vi "Process.vi"(8 "error in":errorcluster, 11 "Plugin in":refnum<class "Nominal-Streamer.lvclass">) -> (0 "error out":errorcluster, 3 "Plugin out":refnum<class "Nominal-Streamer.lvclass">)   [LabVIEW 2020, in "Nominal-Streamer.lvlib" / "Nominal-Streamer.lvclass"]
doc: "Handles incoming data from NI FlexLogger (R) and forwards it to the async processing function."
uses:
  Nominal-Streamer.lvclass
  Nominal-Streamer.lvclass/Nominal-Streamer.ctl
  <vilib>/FlexLogger/SDK/PluginSDK.lvlibp/PEFClasses/SDK/Plugin/Plugin.lvclass
  async queue data.ctl
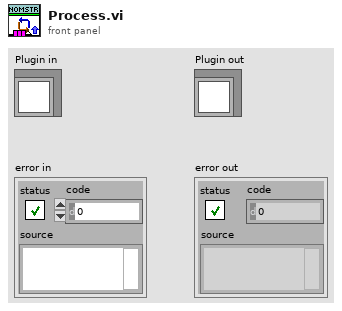
[diagram p1: front panel]
types:
  T1 = typedef "Nominal-Streamer.lvlib/Nominal-Streamer.lvclass/async queue data.ctl" = cluster{"data values":waveform(dbl)[], "data names":string[]}
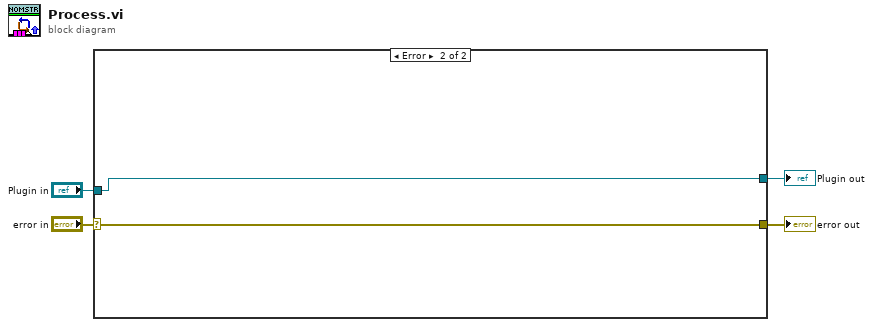
[diagram p0: block diagram]
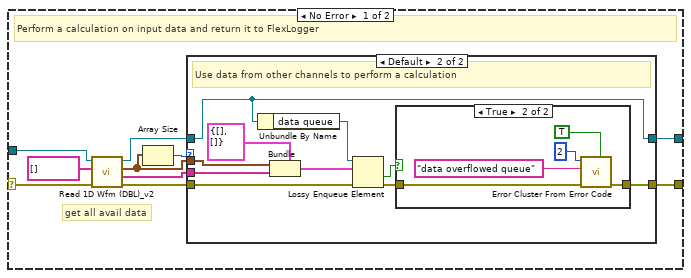
[diagram p2: hidden frame]
diagram:
  n1 = case shown="Error" "error in" {
    selector: "error in" -> [w13 w33]
    tunnel: [w5 w34] -> w1
    tunnel: "Plugin in" -> [w14 w34]
    tunnel: [w12 w33] -> w2
    frame No Error {
      # "get all avail data"
      # "Perform a calculation on input data and return it to FlexLogger"
      n2 = call <vilib>:"Read 1D Wfm (DBL)_v2.vi"("error in (no error)"=w13, "Unique Identifiers (empty = all)"=string[] [] ("Unique Channel Identifers (empty = all)"), "Plugin in"=w14) -> ("error out"=w8:errorcluster, "Stream Names"=w6:string[], "Data"=w11:waveform(dbl)[], "Plugin out"=w9:refnum<class "Nominal-Streamer.lvclass">)  [unwired: 5 in]
      n3 = Array Size(array=w11) -> (size(s)=w10:i32)
      n4 = case shown="Default" w10 {
        tunnel: w11 -> [_ w20]
        tunnel: [w15 w23] -> w12
        tunnel: [w16 w25] -> w5
        tunnel: w9 -> [w16 w25]
        tunnel: w8 -> [w15 w26]
        tunnel: w6 -> [_ w19]
        frame 0 {
          # "this case is used as a sentinel, make sure we don't send!"
          # "No channels sending data to the plugin"
        }
        frame Default {
          # "Use data from other channels to perform a calculation"
          n5 = Unbundle By Name(w25) -> ("data queue"=w21:refnum<queue>)
          n6 = Bundle(cluster=T1 {"data values"=[], "data names"=[]} ("stream data"), "data values"=w20, "data names"=w19) -> (w18:T1)
          n7 = Lossy Enqueue Element(queue=w21, element=w18, error in (no error)=w26) -> (overflow?=w22:bool, error out=w24:errorcluster)  [unwired: 2 out]
          n8 = case shown="True" w22 {
            tunnel: w24 -> [w27 w32]
            tunnel: [w27 w31] -> w23
            frame False {
            }
            frame True {
              n9 = call <vilib>:"Error Cluster From Error Code.vi"("is warning? (False)"=TRUE, "error in (no error)"=w32, "error message (\"\")"="data overflowed queue" ("error message (\"\")"), "error code (0)"=2) -> ("error out"=w31:errorcluster)  [unwired: 5 in]
            }
          }
        }
      }
    }
    frame Error {
    }
  }
  "error out" <- w2
  "Plugin out" <- w1
